vi "Send Schedules to Monkeys.vi"(8 "error in (no error)":errorcluster, 9 "Schedules":refnum<class "Schedule.lvclass">[](array[class]), 10 "Sync. Mask":T1[](array[typedef]), 11 "Tamer in":refnum<class "Tamer.lvclass">) -> (0 "error out":errorcluster, 3 "Tamer out":refnum<class "Tamer.lvclass">)   [LabVIEW 2020, in "Tamer.lvlib" / "Tamer.lvclass"]
uses:
  Tamer.lvclass
  Run Utilities/TypeDefs/Synchronize FPGA Cluster.ctl
  Run Utilities/Schedule/Schedule.lvclass
  C:/LabVIEW Code/CIRCUS/TALOS/TALOS_PPL.lvlibp/Ancestor/Ancestor/Ancestor.lvclass
  TALOS/TALOS_PPL.lvlibp/Guardian/Guardian/Requests.ctl
  Run Utilities/TypeDefs/Messages/Schedule Message.ctl
  Run Utilities/TypeDefs/DAQ Control.ctl
  Run Utilities/TypeDefs/Monkey Status.ctl
  TALOS/TALOS_PPL.lvlibp/Ancestor/Ancestor/Read ID.vi
  Tamer.lvclass/Tamer.ctl
  TALOS/TALOS_PPL.lvlibp/Father of all uServices/Father of all uServices/Father of all uServices.lvclass
  TALOS/TALOS_PPL.lvlibp/Guardian/Guardian/Guardian.lvclass
  Run Utilities/Run Utilities.lvlib
  C:/LabVIEW Code/CIRCUS/TALOS/TALOS_PPL.lvlibp/Father of all uServices/Father of all uServices/Father of all uServices.lvclass
  C:/LabVIEW Code/CIRCUS/TALOS/Actor Framework.lvlibp/1abvi3w/vi.lib/ActorFramework/Actor/Actor.lvclass
  C:/LabVIEW Code/CIRCUS/CIRCUS uServices et al/Tamer/Tamer.lvclass
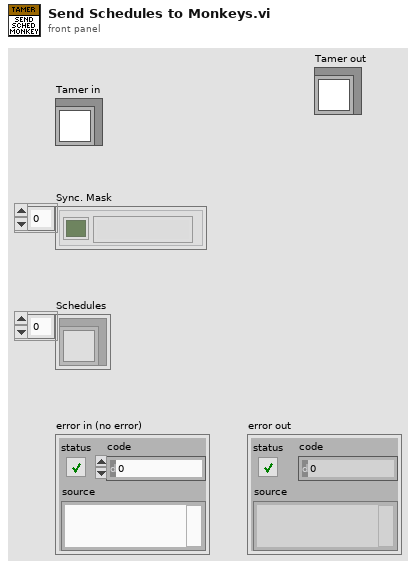
[diagram p1: front panel]
types:
  T1 = typedef "Run Utilities.lvlib/Synchronize FPGA Cluster.ctl" = cluster{"Status":bool, "FPGA Name":string}
  T2 = typedef "TALOS_PPL.lvlibp/Guardian.lvlib/Guardian.lvclass/Requests.ctl" = enum16{"Ready to Launch", "Start RUN", "Stop RUN", "Update DAQ Params", "Update Error Listbox", "Update Run Status", "Update Kasli Log", "Run Stopped with Errors", "Switch uS View"}
  T3 = typedef "Run Utilities.lvlib/Schedule Message.ctl" = cluster{"uS Name":string, "Synchronised":bool, "DAQ Control":T4, "Schedule":refnum<class "Schedule.lvclass">, "Append to top?":bool}
  T4 = typedef "Run Utilities.lvlib/DAQ Control.ctl" = enum16{"On", "Off", "External"}
  T5 = typedef "Run Utilities.lvlib/Monkey Status.ctl" = enum16{"Init", "Paused", "Ongoing", "Stopped", "Finished (no errors)", "Finished (with errors)"}
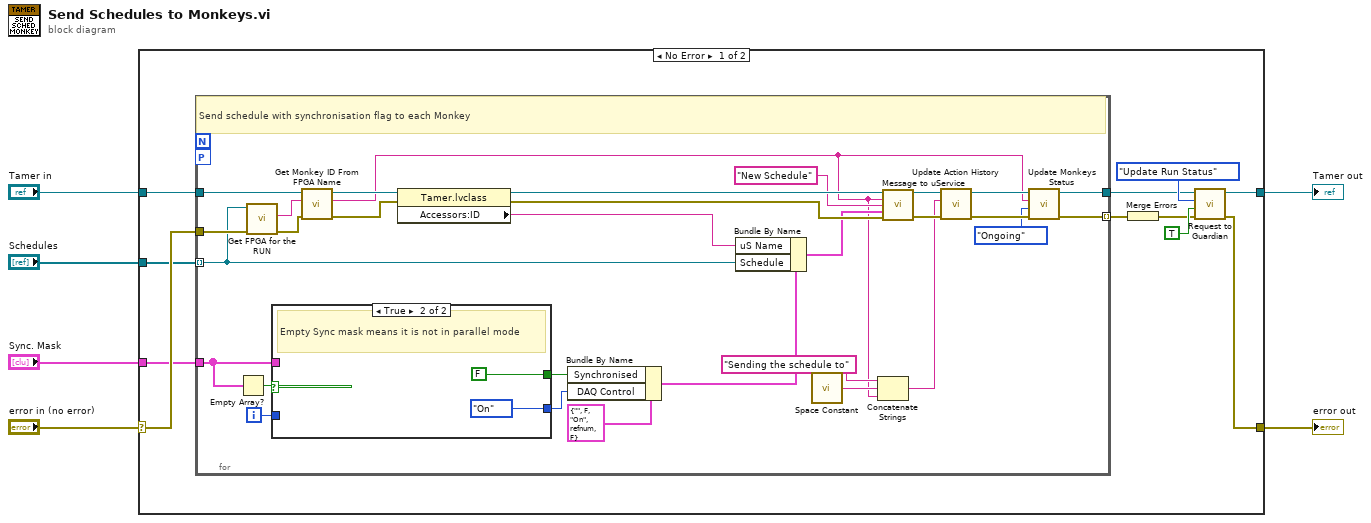
[diagram p0: block diagram]
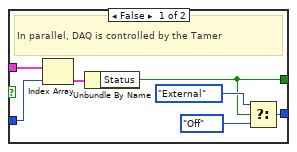
[diagram p2: hidden frame]
diagram:
  n1 = case shown="No Error" "error in (no error)" {
    selector: "error in (no error)" -> [w17 w58]
    tunnel: "Sync. Mask" -> [w16 _]
    tunnel: "Schedules" -> [w15 _]
    tunnel: "Tamer in" -> [w14 w57]
    tunnel: [w10 w58] -> w2
    tunnel: [w9 w57] -> w1
    frame No Error {
      n2 = for {
        tunnel: w14 -> [w33]
        tunnel: w15 -> [w22] mode=indexing
        tunnel: [w25] -> w8 mode=indexing
        tunnel: w16 -> [w41]
        tunnel: [w24] -> w11
        tunnel: w17 -> [w34]
        workers-P: _ -> [_]
        i -> [w42]
        # "Send schedule with synchronisation flag to each Monkey"
        n3 = Empty Array?(array=w41) -> (empty?=w43:bool)
        n4 = call-dynamic "Get FPGA for the RUN.vi"("error in (no error)"=w34, "Schedule in"=w22) -> ("error out"=w30:errorcluster, "FPGA Name"=w31:string)  [unwired: 7 in, 1 out]
        n5 = case shown="True" w43 {
          tunnel: [w48 FALSE] -> w19
          tunnel: w42 -> [w53 _]
          tunnel: w41 -> [w54 _]
          tunnel: [w51 DAQ_Control."On" ("DAQ Control")] -> w20
          frame False {
            # "In parallel, DAQ is controlled by the Tamer"
            n6 = Index Array(array=w54, index=w53) -> (element=w52:T1)
            n7 = Unbundle By Name(w52) -> ("Status"=w48:bool)
            n8 = Select(t=DAQ_Control."External" ("DAQ Control"), s=w48, f=DAQ_Control."Off") -> (s? t:f=w51:T4)
          }
          frame True {
            # "Empty Sync mask means it is not in parallel mode"
          }
        }
        n9 = call-dynamic "Get Monkey ID From FPGA Name.vi"("error in (no error)"=w30, "FPGA Name"=w31, "Tamer in"=w33) -> ("error out"=w29:errorcluster, "Monkey ID"=w26:string, "Tamer out"=w32:refnum<class "Tamer.lvclass">)  [unwired: 6 in]
        n10 = property class="Tamer.lvclass"(reference=w32, error in=w29) -> (reference out=w45:refnum<class "Tamer.lvclass">, error out=w47:errorcluster, "Accessors:ID"=w44:string)
        n11 = Bundle By Name(cluster=T3 {"uS Name"="", "Synchronised"=FALSE, "DAQ Control"=enum."On", "Schedule"=refnum, "Append to top?"=FALSE} ("Monkey Schedule Message"), "Synchronised"=w19, "DAQ Control"=w20) -> (w18:T3)
        n12 = Bundle By Name(cluster=w18, "uS Name"=w44, "Schedule"=w22) -> (w46:T3)
        n13 = call <vilib>:"Space Constant.vi"() -> ("String"=w36:string)
        n14 = Concatenate Strings("Sending the schedule to" ("string"), w36, w26) -> (w38:string)
        n15 = call "Message to uService.vi"("Father of all uServices in"=w45, "uService ID"=w26, "Message"="New Schedule", "Data"=w46, "error in (no error)"=w47) -> ("Father of all uServices out"=w40:refnum<class "Tamer.lvclass">, "error out"=w39:errorcluster)  [unwired: 9 in]
        n16 = call-dynamic "Update Action History.vi"("error in (no error)"=w39, "Action"=w38, "Tamer in"=w40) -> ("error out"=w27:errorcluster, "Tamer out"=w28:refnum<class "Tamer.lvclass">)  [unwired: 7 in]
        n17 = call-dynamic "Update Monkeys Status.vi"("error in (no error)"=w27, "Status"=Monkey_Status."Ongoing", "Monkey ID"=w26, "Tamer in"=w28) -> ("error out"=w25:errorcluster, "Tamer out"=w24:refnum<class "Tamer.lvclass">)  [unwired: 6 in]
      }
      n18 = Merge Errors(w8) -> (w7:errorcluster)
      n19 = call "Request to Guardian.vi"("error in (no error)"=w7, "Data"=TRUE, "Requests"=Requests."Update Run Status", "Father of all uServices in"=w11) -> ("error out"=w10:errorcluster, "Father of all uServices out"=w9:refnum<class "Tamer.lvclass">)  [unwired: 6 in]
    }
    frame Error {
    }
  }
  "error out" <- w2
  "Tamer out" <- w1
